vi "Assert Attach Failed.vi"(8 "error in":errorcluster, 11 "attach error code":i32=-1074097750) -> (0 "error out":errorcluster, 2 "result":string, 3 "pass?":bool)   [LabVIEW 2021, in "MeasurementServerTests.lvlib"]
uses:
  MeasurementServerTests.lvlib
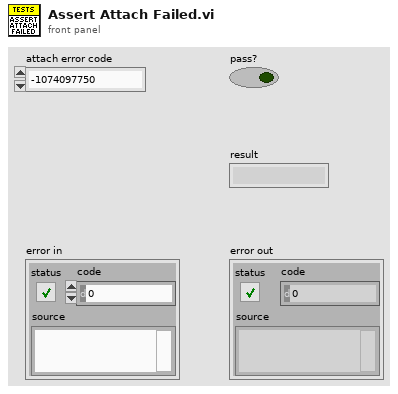
[diagram p1: front panel]
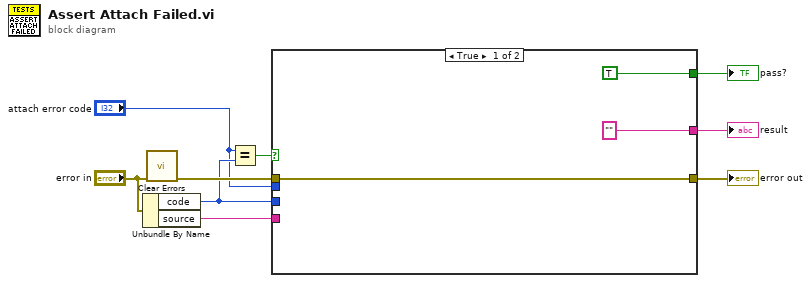
[diagram p0: block diagram]
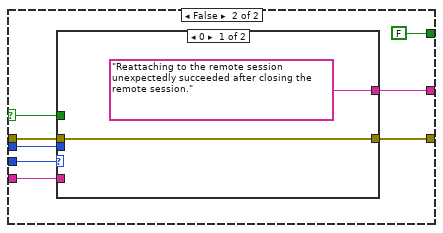
[diagram p2: hidden frame]
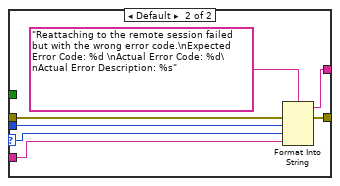
[diagram p3: hidden frame]
diagram:
  n1 = Unbundle By Name("error in") -> ("code"=w2:i32, "source"=w4:string)
  n2 = call <vilib>:"Clear Errors.vi"("error in (no error)"="error in") -> ("error out"=w7:errorcluster)  [unwired: 5 in, 1 out]
  n3 = Equal?(x="attach error code", y=w2) -> (x = y?=w3:bool)
  n4 = case shown="True" w3 {
    selector: w3 -> [_ w20]
    tunnel: ["" ("f") w19] -> w9
    tunnel: [TRUE FALSE] -> w5
    tunnel: w7 -> [w10 w17]
    tunnel: [w10 w16] -> w8
    tunnel: w4 -> [_ w15]
    tunnel: w2 -> [_ w14]
    tunnel: "attach error code" -> [_ w13]
    frame True {
    }
    frame False {
      n5 = case shown="0" w14 {
        selector: w14 -> [_ w24]
        tunnel: w20 -> [_ _]
        tunnel: ["Reattaching to the remote session unexpectedly succeeded after closing the remote session." ("f") w28] -> w19
        tunnel: w17 -> [w21 w27]
        tunnel: [w21 w26] -> w16
        tunnel: w15 -> [_ w23]
        tunnel: w13 -> [_ w25]
        frame 0 {
        }
        frame Default {
          n6 = Format Into String(format string="Reattaching to the remote session failed but with the wrong error code.\nExpected Error Code: %d \nActual Error Code: %d\nActual Error Description: %s" ("f"), error in=w27, w25, w24, w23) -> (resulting string=w28:string, error out=w26:errorcluster)  [unwired: 1 in]
        }
      }
    }
  }
  "result" <- w9
  "error out" <- w8
  "pass?" <- w5
